vi "VIH Constant - VIHelpeks Starter EXE File.vi"() -> (2 "Registry Keys":T1, 3 "VIHelpeks Starter EXE path":path, 5 "In LV Folder":bool)   [LabVIEW 2014]
doc: "::: VI Helpeks :::\nCopyright (c) 2000-2026 Konstantin Shifershteyn. All rights reserved."
panel:
  # "VI Helpeks\nCopyright (c) 2012-2026 Konstantin Shifershteyn"
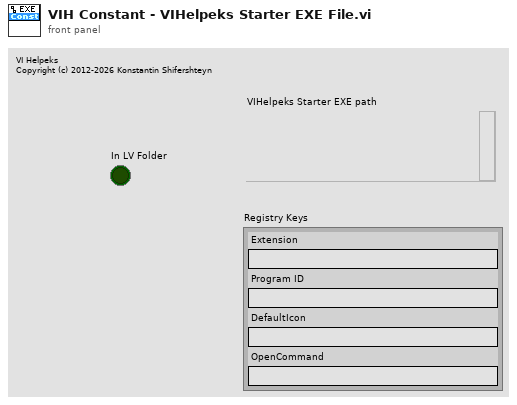
[diagram p1: front panel]
types:
  T1 = cluster{"Extension":string, "Program ID":string, "DefaultIcon":string, "OpenCommand":string}
  T2 = cluster{"Extension":string, "Extension Value":string, "DefaultIcon":string, "OpenCommand":string}
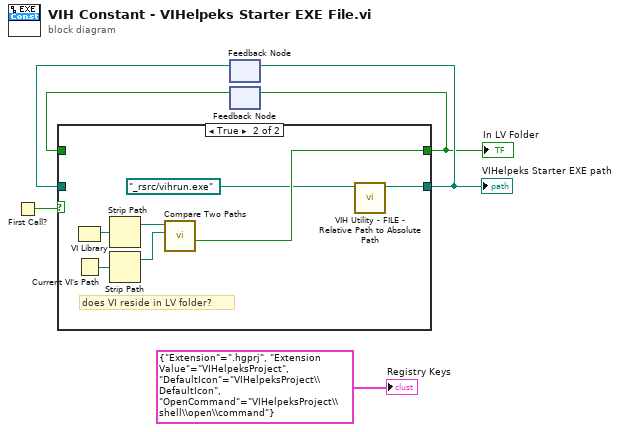
[diagram p0: block diagram]
diagram:
  n1 = First Call?() -> (First Call?: T/F=w6:bool)
  n2 = feedback #1() -> (w5:path)  [unwired: 1 in]
  n3 = feedback #2() -> (w2:bool)  [unwired: 1 in]
  n4 = case shown="True" w6 {
    tunnel: [w8 w15] -> w4
    tunnel: w5 -> [w8 _]
    tunnel: [w7 w10] -> w1
    tunnel: w2 -> [w7 _]
    frame False {
    }
    frame True {
      # "does VI reside in LV folder?"
      n5 = VI Library() -> (path=w11:path)
      n6 = Current VI's Path() -> (path=w14:path)
      n7 = Strip Path(path=w11) -> (stripped path=w12:path)  [unwired: 1 out]
      n8 = Strip Path(path=w14) -> (stripped path=w13:path)  [unwired: 1 out]
      n9 = call <vilib>:"Compare Two Paths.vi"("Path 2"=w13, "Path 1"=w12) -> ("Path 2 Relative to Path 1?"=w10:bool)  [unwired: 6 in, 3 out]
      n10 = call "VIH Utility - FILE - Relative Path to Absolute Path.vi"("Path"=path "_rsrc/vihrun.exe" ("Template HHP File")) -> ("Path out"=w15:path)  [unwired: 9 in, 1 out]
    }
  }
  "VIHelpeks Starter EXE path" <- w4
  "In LV Folder" <- w1
  n11 = feedback-in #1(w4) -> ()
  n12 = feedback-in #2(w1) -> ()
  "Registry Keys" <- T2 {"Extension"=".hgprj", "Extension Value"="VIHelpeksProject", "DefaultIcon"="VIHelpeksProject\\DefaultIcon", "OpenCommand"="VIHelpeksProject\\shell\\open\\command"} ("Registry Keys")
